vi "Pause Unpause.vi"(8 "error in":errorcluster, 11 "PauseUnpause Ref":refnum<vi>) -> (0 "error out":errorcluster, 3 "New Data":string[][](array[string]))   [LabVIEW 2025, in "Automotive Ethernet Bus Monitor UI.lvlib"]
doc: "Returning the new captured data when unpaused. During pause and error returns an empty array."
uses:
  Automotive Ethernet Bus Monitor UI.lvlib
  Table Buffer/Dequeue Data.vi
  Table Buffer/Get Status.vi
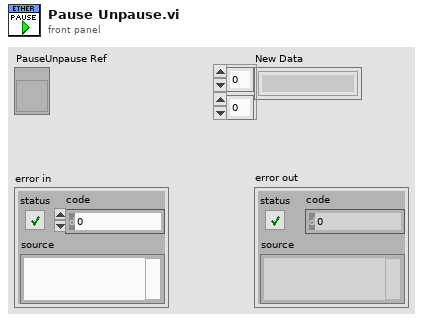
[diagram p1: front panel]
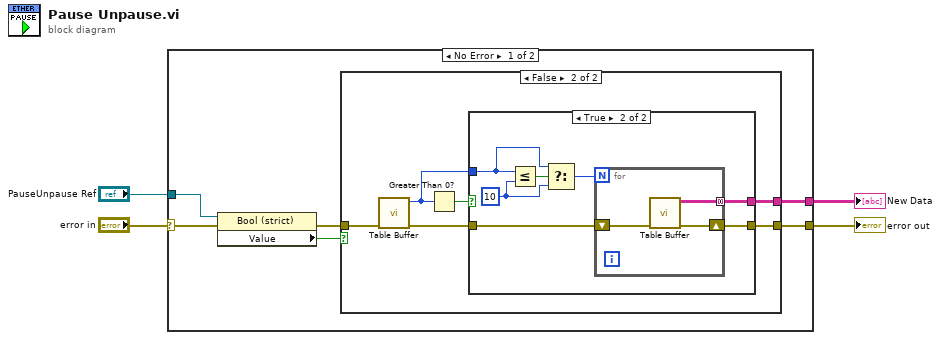
[diagram p0: block diagram]
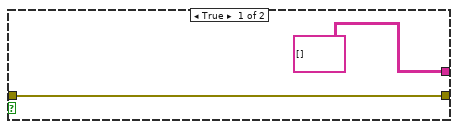
[diagram p2: hidden frame]
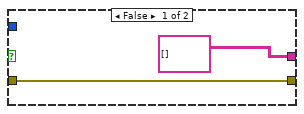
[diagram p3: hidden frame]
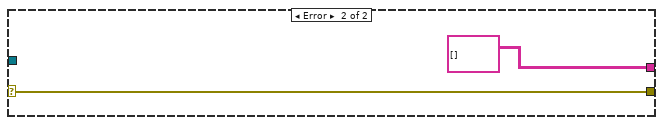
[diagram p4: hidden frame]
diagram:
  n1 = case shown="No Error" "error in" {
    selector: "error in" -> [w5 w32]
    tunnel: [w10 string[][] [] ("Dataframe 3")] -> w4
    tunnel: "PauseUnpause Ref" -> [w7 _]
    tunnel: [w6 w32] -> w2
    frame No Error {
      n2 = property class="Bool (strict)"(reference=w7, error in=w5) -> (error out=w9:errorcluster, "Value"=w8:bool)  [unwired: 1 out]
      n3 = case shown="False" w8 {
        tunnel: w9 -> [w11 w15]
        tunnel: [string[][] [] ("Dataframe 3") w18] -> w10
        tunnel: [w11 w17] -> w6
        frame True {
        }
        frame False {
          n4 = call-poly "Table Buffer.vi"("error in"=w15) -> ("error out"=w16:errorcluster, "Messages"=w13:i32)  [unwired: 9 in]
          n5 = Greater Than 0?(x=w13) -> (x > 0?=w14:bool)
          n6 = case shown="True" w14 {
            tunnel: [string[][] [] ("Data") w27] -> w18
            tunnel: [w20 w26] -> w17
            tunnel: w16 -> [w20 w25]
            tunnel: w13 -> [_ w22]
            frame False {
            }
            frame True {
              w23 = 10 ("y")
              n7 = Less Or Equal?(x=w22, y=w23) -> (x <= y?=w24:bool)
              n8 = Select(t=w22, s=w24, f=w23) -> (s? t:f=w21:i32)
              n9 = for {
                N: w21 -> [_]
                tunnel: [w30] -> w27 mode=concatenating
                shift-right: [w29] -> w26
                shift-left: w25 -> [w28]
                n10 = call-poly "Table Buffer.vi"("error in"=w28) -> ("error out"=w29:errorcluster, "Data"=w30:string[][])  [unwired: 9 in]
              }
            }
          }
        }
      }
    }
    frame Error {
    }
  }
  "New Data" <- w4
  "error out" <- w2
